vi "VIH ProjFile - Product Info - Write.vi"(8 "error in":errorcluster, 9 "Product Info":T1, 11 "XML Parent Item":refnum<k20>) -> (0 "error out":errorcluster, 3 "dup XML Parent Item":refnum<k20>)   [LabVIEW 2014]
doc: "::: VI Helpeks :::\nCopyright (c) 2000-2026 Konstantin Shifershteyn. All rights reserved."
uses:
  _VIH HelpGen.llb/VIH HelpGen Typedef - Product Info Cluster.ctl
  <vilib>/xml/Close Reference(Node).vi
  <resource>/objmgr/DOMUserDefRef.rc
  <vilib>/xml/NI_XML.lvlib
panel:
  in  "Product Info (data)":T1
  # "VI Helpeks\nCopyright (c) 2012-2026 Konstantin Shifershteyn"
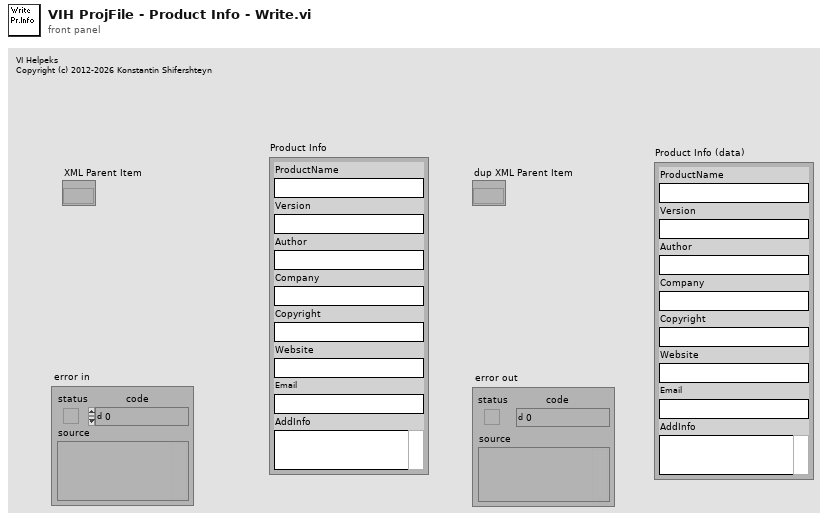
[diagram p1: front panel]
types:
  T1 = typedef "VIH HelpGen Typedef - Product Info Cluster.ctl" = cluster{"ProductName":string, "Version":string, "Author":string, "Company":string, "Copyright":string, "Website":string, "Email":string, "AddInfo":string}
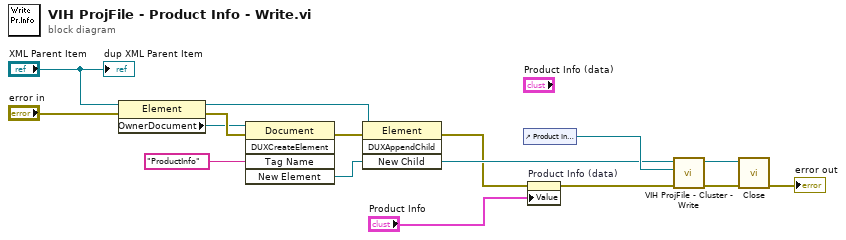
[diagram p0: block diagram]
diagram:
  n1 = property class="Element"(reference="XML Parent Item", error in="error in") -> (reference out=w6:refnum<k20>, error out=w8:errorcluster, "OwnerDocument"=w5:refnum<k20>)
  n2 = invoke class="Document" method="DUXCreateElement"(reference=w5, error in=w8, "Tag Name"="ProductInfo") -> (error out=w10:errorcluster, "New Element"=w14:refnum<k20>)  [unwired: 2 in, 3 out]
  n3 = invoke class="Element" method="DUXAppendChild"(reference=w6, error in=w10, "New Child"=w14) -> (error out=w12:errorcluster)  [unwired: 1 in, 3 out]
  n4 = control-ref of="Product Info (data)"() -> (w15:refnum<vi>)
  n5 = property on="Product Info (data)" class="Clust (strict)"(error in=w12, "Value"="Product Info") -> (error out=w13:errorcluster)  [unwired: 1 in, 1 out]
  n6 = call "VIH ProjFile - Cluster - Write.vi"("error in"=w13, "Ctl Refnum"=w15, "XML Parent Item"=w14) -> ("error out"=w2:errorcluster, "dup XML Parent Item"=w3:refnum<k20>)  [unwired: 7 in]
  n7 = call-poly <vilib>:"Close.vi"("error in (no error)"=w2, "node"=w3) -> ("error out"=→"error out":errorcluster)  [unwired: 7 in]
  "dup XML Parent Item" <- "XML Parent Item"
